vi "Test Addition.vi"(8 "error in (no error)":errorcluster) -> (0 "error out":errorcluster)   [LabVIEW 2020]
doc: "This is an example test case."
uses:
  classes/Properties.Assert/Properties.Assert.lvclass
  C:/projects/caraya/src/classes/Properties/Properties.lvclass
  classes/Test/Test.lvclass
  classes/Assert/Assert.lvclass
  classes/Properties/Properties.lvclass
panel:
  # "See block diagram"
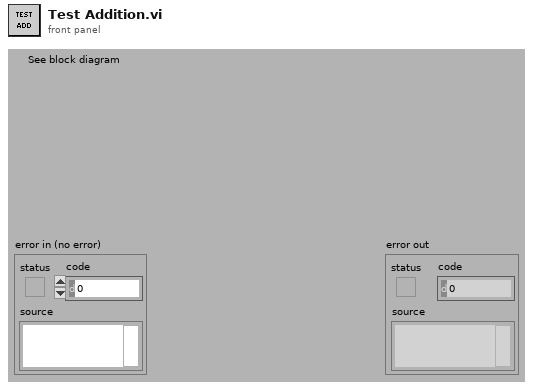
[diagram p1: front panel]
types:
  T1 = cluster{"Requirement ID":string, "Requirement ID":string}
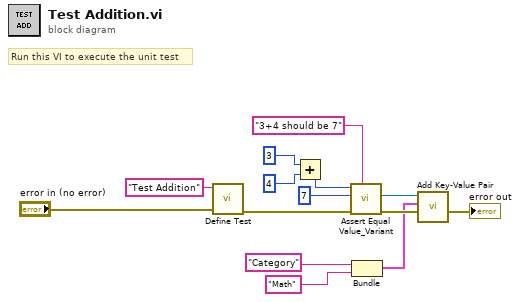
[diagram p0: block diagram]
diagram:
  # "Run this VI to execute the unit test"
  n1 = call "Define Test.vi"("error in (no error)"="error in (no error)", "Label (VI Title)"="Test Addition") -> ("error out"=w10:errorcluster)  [unwired: 8 in, 1 out]
  n2 = Add(x=3, y=4) -> (x+y=w8:i32)
  n3 = call "Assert Equal Value_Variant.vi"("Label"="3+4 should be 7", "error in (no error)"=w10, "Y"=7, "X"=w8) -> ("error out"=w5:errorcluster, "Properties.Assert"=w6:refnum<class "Properties.Assert.lvclass">)  [unwired: 6 in]
  n4 = Bundle("Requirement ID"="Category", "Requirement ID"="Math") -> (w2:T1)  [unwired: 1 in]
  n5 = call "Add Key-Value Pair.vi"("error in (no error)"=w5, "entry"=w2, "Properties in"=w6) -> ("error out"=→"error out":errorcluster)  [unwired: 7 in, 1 out]
